vi "Disable.vi"(11 "logger in":refnum<class "Logger.lvclass">) -> (3 "logger out":refnum<class "Logger.lvclass">)   [LabVIEW 2018, in "GLog.lvlib" / "Logger.lvclass"]
uses:
  Logger.lvclass
  Logger.lvclass/Logger.ctl
panel:
  # "Connector Pane"
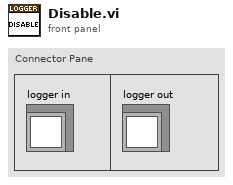
[diagram p1: front panel]
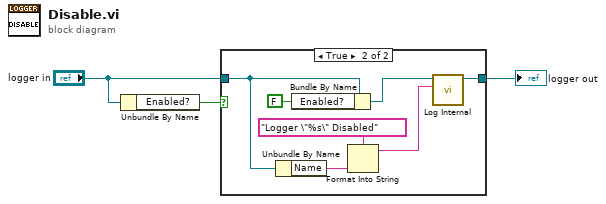
[diagram p0: block diagram]
diagram:
  n1 = Unbundle By Name("logger in") -> ("Enabled?"=w1:bool)
  n2 = case shown="True" w1 {
    tunnel: "logger in" -> [w4 w5]
    tunnel: [w4 w6] -> w3
    frame False {
    }
    frame True {
      n3 = Unbundle By Name(w5) -> ("Name"=w10:string)
      n4 = Bundle By Name(cluster=w5, "Enabled?"=FALSE) -> (w7:refnum<class "Logger.lvclass">)
      n5 = Format Into String(format string="Logger \"%s\" Disabled" ("message"), w10) -> (resulting string=w8:string)  [unwired: 2 in, 1 out]
      n6 = call "Log Internal.vi"("message"=w8, "logger in"=w7) -> ("logger out"=w6:refnum<class "Logger.lvclass">)  [unwired: 9 in]
    }
  }
  "logger out" <- w3
